vi "Test_Render.vi"() -> ()   [LabVIEW 2026]
doc: "UI_Render_Main 테스트 (PNG 경로 필수)."
panel:
  out "error out":errorcluster
  in  "PNG Path":path
  in  "Running":bool=TRUE
  in  "Phase":bool=TRUE
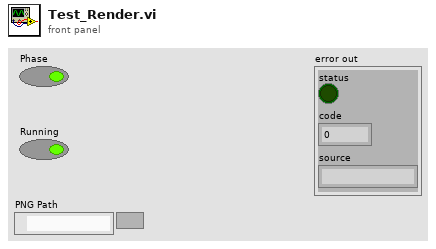
[diagram p1: front panel]
types:
  T1 = cluster{"left":i16, "top":i16, "right":i16, "bottom":i16}
  T2 = cluster{"Name":string, "Value":dbl, "High Limit":dbl, "Low Limit":dbl, "Save":bool, "Graph":bool, "Scale Min":dbl, "Scale Max":dbl, "Unit":string}[]
  T3 = cluster{"Name":string, "Value":dbl, "High Limit":dbl, "Low Limit":dbl, "Save":bool, "Graph":bool, "Scale Min":dbl, "Scale Max":dbl, "Unit":string}
  T4 = typedef "imagedata.ctl" = cluster{"image type":i32, "image depth":i32, "image":u8[], "mask":u8[], "colors":u32[], "Rectangle":cluster{"left":i16, "top":i16, "right":i16, "bottom":i16}}
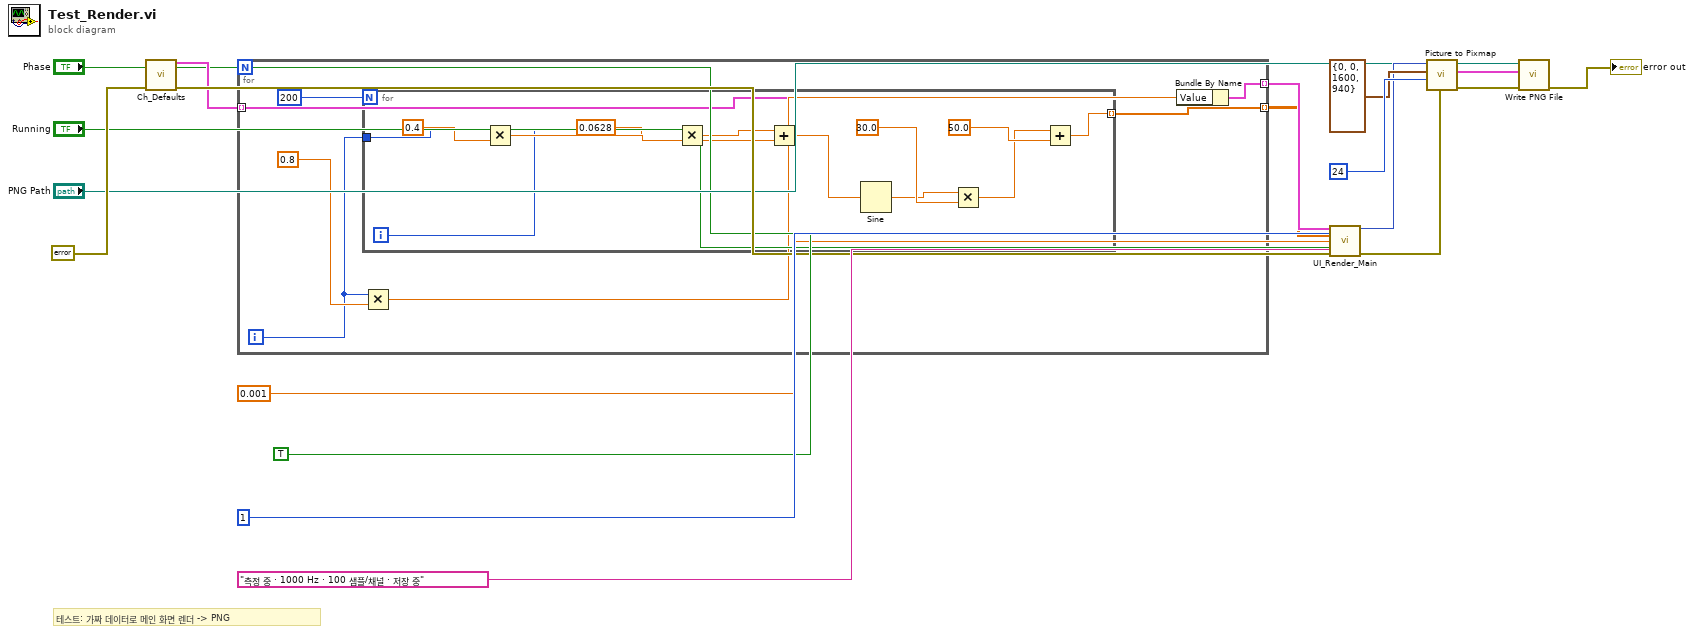
[diagram p0: block diagram]
diagram:
  # "테스트: 가짜 데이터로 메인 화면 렌더 -> PNG"
  n1 = call "Ch_Defaults.vi"("error in"=errorcluster {"status"=FALSE, "code"=0, "source"=""}) -> ("Channels"=w5:T2, "error out"=w6:errorcluster)  [unwired: 13 in]
  n2 = for {
    tunnel: w5 -> [w20] mode=indexing
    tunnel: [w25] -> w8 mode=indexing
    tunnel: [w22] -> w7 mode=indexing
    i -> [w19]
    n3 = for {
      N: 200 -> [_]
      tunnel: w19 -> [w27]
      tunnel: [w37] -> w22 mode=indexing
      i -> [w26]
      n4 = Multiply(x=w27, y=0.4) -> (x*y=w31:dbl)
      n5 = Multiply(x=w26, y=0.0628) -> (x*y=w29:dbl)
      n6 = Add(x=w29, y=w31) -> (x+y=w32:dbl)
      n7 = Sine(x=w32) -> (sin(x)=w33:dbl)
      n8 = Multiply(x=w33, y=30.0) -> (x*y=w35:dbl)
      n9 = Add(x=w35, y=50.0) -> (x+y=w37:dbl)
    }
    n10 = Multiply(x=w19, y=0.8) -> (x*y=w24:dbl)
    n11 = Bundle By Name(cluster=w20, "Value"=w24) -> (w25:T3)
  }
  n12 = call "UI_Render_Main.vi"("Channels"=w8, "Logging"=TRUE, "Hover Button"=1, "Phase"="Phase", "Data"=w7, "dt"=0.001, "Running"="Running", "error in"=w6, "Status"="측정 중 · 1000 Hz · 100 샘플/채널 · 저장 중") -> ("Picture"=w13:picture, "error out"=w14:errorcluster)  [unwired: 5 in]
  n13 = call <vilib>:"Picture to Pixmap.vi"("depth"=24, "rect"=T1 {"left"=0, "top"=0, "right"=1600, "bottom"=940}, "picture"=w13) -> ("image data"=w17:T4)  [unwired: 7 in, 1 out]
  n14 = call <vilib>:"Write PNG File.vi"("error in (no error)"=w14, "image data"=w17, "path to PNG file"="PNG Path") -> ("error out"=→"error out":errorcluster)  [unwired: 7 in, 1 out]
